vi "_ExponentialCalculation.vi"(1 "Initial FP:Transparency":u8) -> (0 "Transparency Array":u8[](array[numeric]))   [LabVIEW 2012]
doc: "Calculates the exponential gradient and returns an array of percentages."
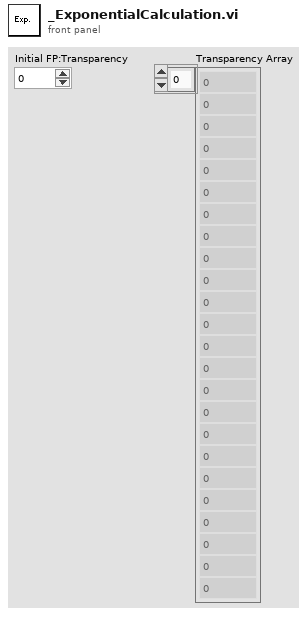
[diagram p1: front panel]
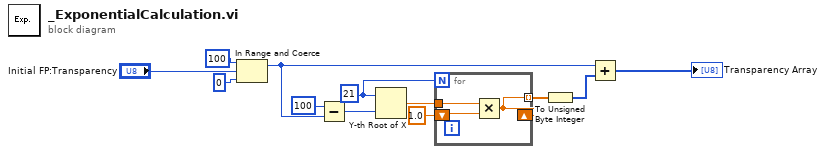
[diagram p0: block diagram]
diagram:
  w8 = 21
  n1 = In Range and Coerce(upper limit=u8 100, x="Initial FP:Transparency", lower limit=u8 0) -> (coerced(x)=w1:u8)  [unwired: 1 out]
  n2 = Subtract(x=u8 100, y=w1) -> (x-y=w10:u8)
  n3 = Y-th Root of X(1:w10, 2:w8) -> (0:w5:dbl)
  n4 = for {
    N: w8 -> [_]
    shift-right: [w13] -> _
    shift-left: 1.0 -> [w14]
    tunnel: w5 -> [w15]
    tunnel: [w13] -> w7 mode=indexing
    n5 = Multiply(x=w15, y=w14) -> (x*y=w13:dbl)
  }
  n6 = To Unsigned Byte Integer(number=w7) -> (unsigned 8bit integer=w11:u8[])
  n7 = Add(x=w1, y=w11) -> (x+y=→"Transparency Array":u8[])
